vi "Run - API Logging PWP (SubVI).vi"(8 "error in (no error)":errorcluster, 10 "Elapse Time":string, 11 "Cluster":T1 {"M Event" items=["Stop", "Running", "PID", "Up Limit", "Down Limit", "Load Limit"]; "Test Type" items=["Please Select"=0, "Triaxial Shear"=1, "Triaxial UU"=2, "Shearbox"=3, "Permeability"=4, "Consolidation (Stepped Loading)/Swelling"=5, "UCT"=8, "Isotropic Consolidation"=9, "Swelling Pressure"=10, "B-Check"=11, "Saturation (Step Increment)"=12, "Saturation (Ramp)"=13]; "Data"."Test Type" items=["Please Select"=0, "Triaxial Shear"=1, "Triaxial UU"=2, "Shearbox"=3, "Permeability"=4, "Consolidation (Stepped Loading)/Swelling"=5, "UCT"=8, "Isotropic Consolidation"=9, "Swelling Pressure"=10, "B-Check"=11, "Saturation (Step Increment)"=12, "Saturation (Ramp)"=13]}) -> (0 "error out":errorcluster, 1 "JSON string":string, 2 "body":string, 3 "Cluster 2":T1 {"M Event" items=["Stop", "Running", "PID", "Up Limit", "Down Limit", "Load Limit"]; "Test Type" items=["Please Select"=0, "Triaxial Shear"=1, "Triaxial UU"=2, "Shearbox"=3, "Permeability"=4, "Consolidation (Stepped Loading)/Swelling"=5, "UCT"=8, "Isotropic Consolidation"=9, "Swelling Pressure"=10, "B-Check"=11, "Saturation (Step Increment)"=12, "Saturation (Ramp)"=13]; "Data"."Test Type" items=["Please Select"=0, "Triaxial Shear"=1, "Triaxial UU"=2, "Shearbox"=3, "Permeability"=4, "Consolidation (Stepped Loading)/Swelling"=5, "UCT"=8, "Isotropic Consolidation"=9, "Swelling Pressure"=10, "B-Check"=11, "Saturation (Step Increment)"=12, "Saturation (Ramp)"=13]})   [LabVIEW 2019]
uses:
  Controls/RunTest - Data Structure.ctl
  Controls/Test Panel - Data Structure.ctl
  Controls/Station - Test Type.ctl
  <vilib>/Utility/miscctls.llb/LVRowAndColumnTypeDef.ctl
  Controls/RunTest - Calculate Data.ctl
  <vilib>/httpClient/ClientHandle.ctl
  Controls/RunTest - Start Condition.ctl
  Controls/RunTest - Stop Condition.ctl
  Controls/UDP - Event.ctl
  <vilib>/httpClient/POSTBuffer.vi
  <vilib>/httpClient/LabVIEWHTTPClient.lvlib
panel:
  out "headers":string
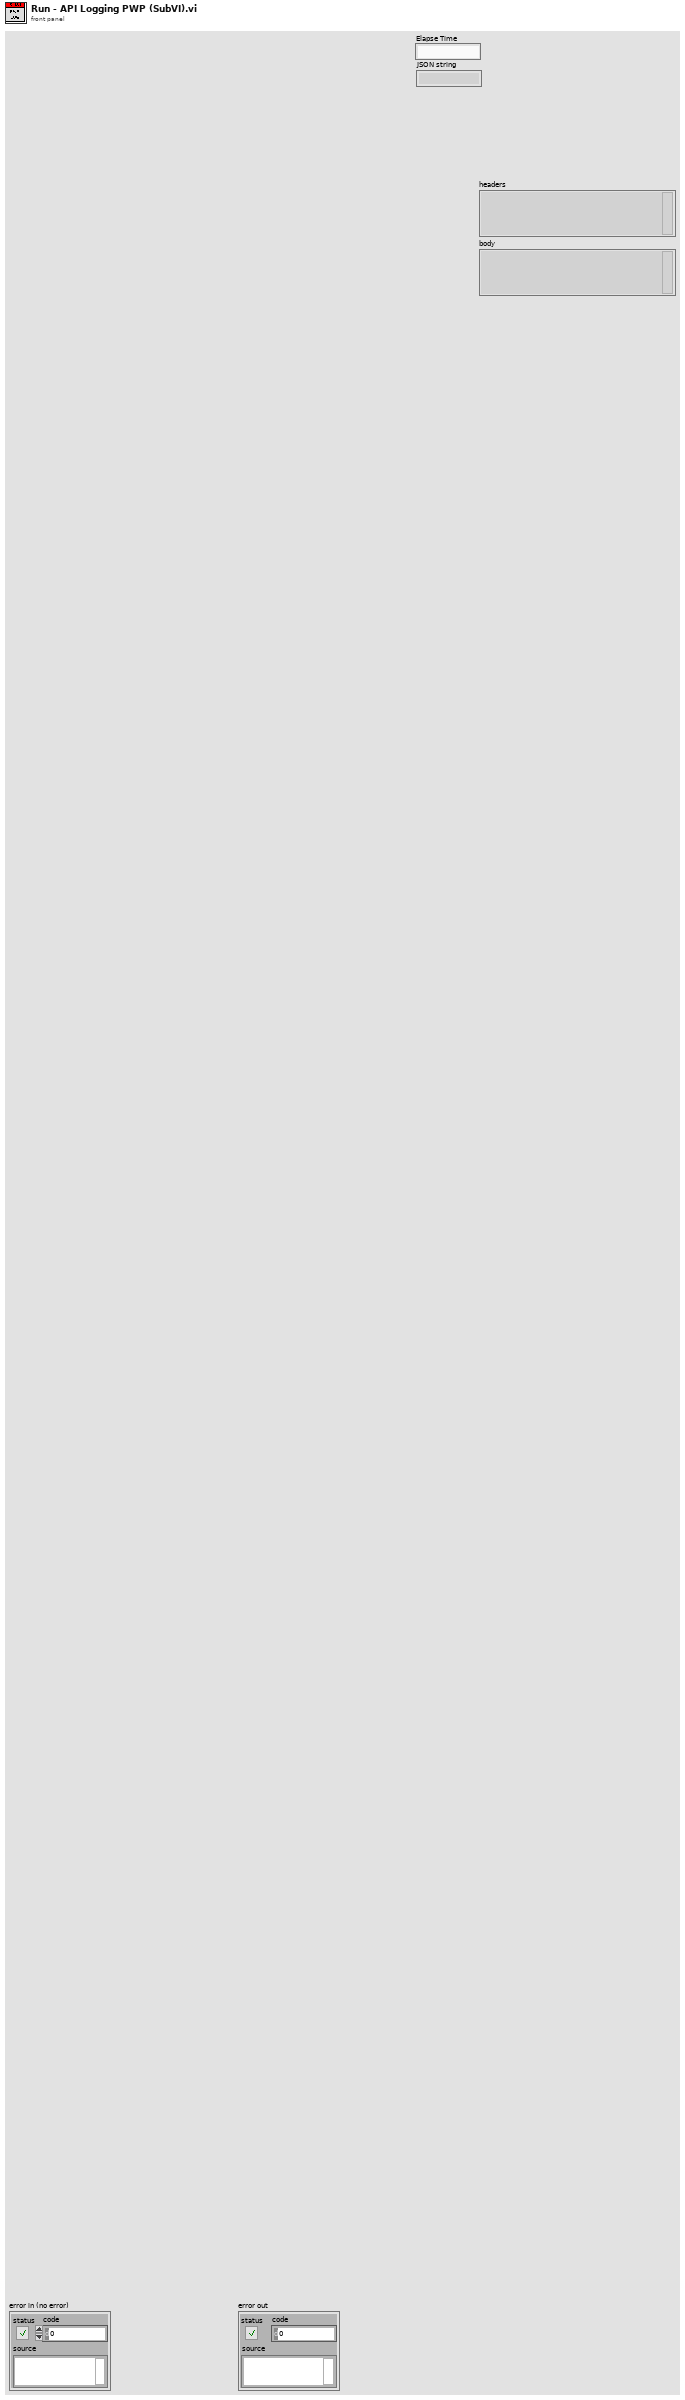
[diagram p1: front panel]
types:
  T1 = typedef "RunTest - Data Structure.ctl" = cluster{"Test Plan":string[], "PlanRow":i32, "Device Name":string[], "Timeout":i32, "Start?":bool, "Pause?":bool, "IP Address":string[], "LogRow":i32, "Logtype":u16, "Log Elapse":sgl, "Data":T2, "Stop log?":bool, "tdms":refnum<k34>, "Sensor Data":sgl[], "Start time":timestamp, "Prev Log Elapse":u32, "Plot":u16, "X-Axis":u16[], "Y-Axis":u16[], "XY":cluster{"X":dbl, "Y":dbl}[][], "End Stage?":bool, "1run":bool, "Condition":u16[], "Start Con":bool, "Log Con":bool, "Stop Con":bool, "Start Elapse":dbl, "Start Load":dbl, "Motor":i32, "StartRow":i32, "number log":i32, "Dir":bool, "Start time test":timestamp, "Auto":bool, "Check return?":bool, "Inv":cluster{"M":i32[], "Bool":bool[]}, "tdms temp":refnum<k34>, "Zero?":bool, "Plot Timer":dbl, "1st Run":bool, "TDMS Path":path, "MaxLoad":dbl, "Log Timer":sgl[], "Test Type":T3, "Log Sensor":string[], "Save?":bool, "1st Log":bool, "Y-Axis 2":u16[], "On Y-Axis 2":bool, "Decimal":u8[], "Init":cluster{"PWP TS":sgl, "Load TS":sgl, "Volume TS":sgl, "Disp TS":sgl, "CP":sgl, "Vol In":sgl, "Vol Out":sgl, "Load UCT":sgl, "Disp UCT":sgl, "PWP Sat":sgl, "CP Sat":sgl, "Volume IsoCons":sgl, "PWP IsoCons":sgl, "PWP TUU":sgl, "Load TUU":sgl, "Volume TUU":sgl, "Disp TUU":sgl, "Load Cons":sgl, "Disp Cons":sgl, "Volume Sat":sgl, "Vertical Load SB":sgl, "Vertical Disp SB":sgl, "H Disp SB":sgl, "H Load SB":sgl, "PWP BC":sgl, "CP BC":sgl, "PWP Sat Step":sgl, "CP Sat Step":sgl, "Volume Sat Step":sgl, "PWP Sat Ramp":sgl, "CP Sat Ramp":sgl, "Volume Sat Ramp":sgl}, "Calc":T5, "Device Index":i32[], "Channel Index":i32[], "http ref":T6, "fileid":string, "Step Cons":cluster{"V Stress":sgl, "H Settlement":sgl}, "RunTest":bool, "Graph Last":i32, "Init?":bool, "Datalog":bool[], "Start":T7, "Stop":T8, "Running?":bool, "StartTime":dbl, "Log Prev Time":dbl, "KeyName":string[], "Test RunTime":dbl, "Log Prev Axial":dbl, "M Event":T9[], "Last Log":bool, "popup":bool, "PreStart UU":bool, "PreStart Sat":bool, "PreStart BC":bool, "PreStart Sat Step":bool, "PreStart Sat Ramp":bool, "Prev Sat IP":string, "IP Device ID":string[]}
  T2 = typedef "Test Panel - Data Structure.ctl" = cluster{"Station":string, "Sample ID":string, "Job No":string, "Job Description":string, "Filename":string, "Test Type":T3, "Speciment No":string, "Depth":string, "Height":string, "Diameter/Length":string, "Weight":string, "Test Parameter":string, "Station[]":string[], "Edit Pos":T4, "Edit Pos Prev":T4, "Area":string, "Path":string, "sample_id":string}
  T3 = typedef "Station - Test Type.ctl" = u16
  T4 = typedef "LVRowAndColumnTypeDef.ctl" = cluster{"Row":i32, "Column":i32}
  T5 = typedef "RunTest - Calculate Data.ctl" = cluster{"TS":cluster{"Change PWP":sgl, "Change Vol":sgl, "Axial Load":sgl, "CiL":sgl, "Deviator":sgl, "Axial Strain":sgl, "MaxDeviator":sgl, "SS":sgl, "CAS":sgl}, "TUU":cluster{"Change PWP":sgl, "Axial Load":sgl, "CiL":sgl, "Deviator":sgl, "Axial Strain":sgl, "MaxDeviator":sgl}, "Sat":cluster{"B Value":sgl, "PWP Diss":sgl, "CPP":sgl, "CV":sgl}, "Per":cluster{"Change Vol In":sgl, "Change Vol Out":sgl, "Mean Vol":sgl, "Gradient Pressure":sgl, "Outlet Flow":sgl, "Inlet Flow":sgl, "I X1":sgl, "I X2":sgl, "I Y1":sgl, "I Y2":sgl, "O X1":sgl, "O X2":sgl, "O Y1":sgl, "O Y2":sgl}, "Step Cons":cluster{"V Stress":sgl, "H Settlement":sgl, "Total H Settle":sgl, "Prev Total H":sgl}, "UCT":cluster{"ALC":sgl, "H Change":sgl, "Deviator":sgl, "Axial Strain":sgl, "V Stress":sgl, "MaxDeviator":sgl}, "ISO Cons":cluster{"CPP":sgl, "PWP Diss":sgl, "CV":sgl, "VS":sgl}, "SB":cluster{"Speci LenC":sgl, "Shear Strain":sgl, "H LC":sgl, "Normal Stress":sgl, "Shear Stress":sgl, "MaxShear":sgl}, "BC":cluster{"B Value":sgl, "PWP Diss":sgl, "CPP":sgl, "CV":sgl}, "Sat Step":cluster{"B Value":sgl, "PWP Diss":sgl, "CPP":sgl, "CV":sgl}, "Sat Ramp":cluster{"B Value":sgl, "PWP Diss":sgl, "CPP":sgl, "CV":sgl}, "Prev Log":string[]}
  T6 = typedef "LabVIEWHTTPClient.lvlib/ClientHandle.ctl" = refnum<k1>
  T7 = typedef "RunTest - Start Condition.ctl" = cluster{"Cons":cluster{"VS":dbl, "Delay":bool, "No Delay":dbl}, "Sat":cluster{"CP":dbl, "BP":dbl, "StartBP":bool, "Target CP":bool, "Target BP":bool}, "Iso":cluster{"Select":dbl, "BP":dbl, "IC2":dbl, "IC3":dbl, "IC4":dbl, ". IC6":bool, "IC6":dbl, "IC6-2":dbl, "Time Cond":dbl, "Last PWP":dbl, "Target CP":bool, "Target BP":bool, "NewCP":dbl, "NewBP":dbl, "Noti CP":bool, "Noti BP":bool, "Noti PWP":bool, "PrevSatBP":dbl}, "TS":cluster{"SS":dbl, "Engage":bool, "ES":dbl, "LC":dbl, "PreStart":bool, "Trig SS":bool, "Drain":dbl, "Select":u16, "Max SS .":bool, "MaxSS":dbl}, "TUU":cluster{"SS":dbl, "Engage":bool, "ES":dbl, "LC":dbl, "PreStart":bool, "Trig SS":bool, "CP":dbl, "Delay Value":dbl, "Delay":bool, "CP PID":bool}, "UCT":cluster{"SS":dbl, "Engage":bool, "ES":dbl, "LC":dbl, "PreStart":bool, "Trig SS":bool}, "Enable?":bool, "SB":cluster{"SS":dbl, "Engage":bool, "ES":dbl, "LC":dbl, "PreStart":bool, "Trig SS":bool, "VS":dbl, "Delay Value":dbl, "Delay":bool, "VS PID":bool}, "Perm":cluster{"DP":dbl}, "BC":cluster{"CP":dbl, "Target CP":bool, "Target BP":bool, "CP Inc":dbl, "CP .Init":bool, "CP Init":dbl, "1st BC":bool}, "Sat (Step)":cluster{"Select":dbl, "CP":dbl, "BP":dbl, "EP":dbl, "StartCP":bool, "Target CP":bool, "Target BP":bool}, "Sat (Ramp)":cluster{"Select":dbl, "CP":dbl, "BP":dbl, "EP":dbl, "StartCP":bool, "Target CP":bool, "Target BP":bool, "Time Rate":u32}}
  T8 = typedef "RunTest - Stop Condition.ctl" = cluster{"Cons":cluster{"Select":i32, "Disp":dbl, "Time":dbl, "Time2":dbl, "Disp 2":dbl, "Time Cond":dbl, "Last Disp":dbl, "Swell":bool, "T50,90,100":cluster{"t50_x_min":dbl, "t50_y_value":dbl, "t90_x_min":dbl, "t90_y_value":dbl, "t100_x_min":dbl, "t100_y_value":dbl, "target_column":string, "test_type":string, "error":string}}, "Sat":cluster{"Select":i32, "PP":dbl, "Time":dbl, "VC":dbl, "Time2":dbl, "Time Cond":dbl, "Last PP":dbl, ".B":bool, "B":dbl, "Last Vc":dbl, "Time Cond 2":dbl, "Time3":dbl, "Time Cond 3":dbl, "B Achieve":bool, "PP Achieve":bool, "VC Achieve":bool, "Max Achieve":bool, "CP Check":dbl, "Skip Next":bool, "B Achieve Stage":u32, ".CP Check":bool}, "Iso":cluster{"PP":dbl, "Time":dbl, "VC":dbl, "Time2":dbl, "Time Cond":dbl, "Last Vc":dbl, ".PP":bool, "Time Cond 2":dbl, "Select":i32, "BS":cluster{"t50_x_min":dbl, "t50_y_value":dbl, "t90_x_min":dbl, "t90_y_value":dbl, "t100_x_min":dbl, "t100_y_value":dbl, "target_column":string, "test_type":string, "error":string}, "Final VC":dbl, "ASTM":cluster{"t50_x_min":dbl, "t50_y_value":dbl, "t90_x_min":dbl, "t90_y_value":dbl, "t100_x_min":dbl, "t100_y_value":dbl, "target_column":string, "test_type":string, "error":string}, "ASTM Log":cluster{"t50_x_min":dbl, "t50_y_value":dbl, "t90_x_min":dbl, "t90_y_value":dbl, "t100_x_min":dbl, "t100_y_value":dbl, "target_column":string, "test_type":string, "error":string}, "PP Achieve":bool, "VC Achieve":bool}, "TS":cluster{"Axial":dbl, ".MaxDev":bool, "MaxDev Value":dbl, "Return":bool, "Reset":bool, "Prev Time":dbl, "PostStop Run":bool, "CP Stop":bool, "BP Stop":bool, "PostStop Trig":bool, "Reset Value":dbl, "BPTrig":bool, "CPTrig":bool, "VLCTrig":bool, "CAxial":dbl, "Select":i32}, "TUU":cluster{"Axial":dbl, ".MaxDev":bool, "MaxDev Value":dbl, "Return":bool, "Reset":bool, "Prev Time":dbl, "PostStop Run":bool, "CP Stop":bool, "BP Stop":bool, "PostStop Trig":bool, "Reset Value":dbl, "BPTrig":bool, "CPTrig":bool, "VLCTrig":bool}, "UCT":cluster{"Axial":dbl, ".MaxDev":bool, "MaxDev Value":dbl, "Return":bool, "Reset":bool, "Prev Time":dbl, "PostStop Run":bool, "CP Stop":bool, "BP Stop":bool, "PostStop Trig":bool}, "Enable?":bool, "SB":cluster{"Shear":dbl, ".MaxShear":bool, "MaxShear Value":dbl, "Return":bool, "Reset":bool, "Prev Time":dbl, "PostStop Run":bool, "CP Stop":bool, "BP Stop":bool, "PostStop Trig":bool, "Reset Value":dbl, "BPTrig":bool, "CPTrig":bool, "VLCTrig":bool}, "Perm":cluster{"Max Time":bool, "Reset":bool, "PostStop Run":bool, "Ratio":bool, "Reset Value":dbl, "Time":dbl, "RatioTime":dbl, "RatioMore":dbl, "RatioLess":dbl, "Time Cond":dbl, "Time Cond 2":dbl, "Prev IF":dbl, "Prev OF":dbl, "PostStop Trig":bool, "BP Trig":bool, "DP Stop":bool, "BP Stop":bool, "CP Stop":bool, "CP Trig":bool}, "SP":cluster{".Max Time":bool, ".Time":bool, "Time":dbl, "MaxTime":dbl, "Time Cond":dbl, "Max Time Cond":dbl, "Stress":dbl}, "BC":cluster{"Select":i32, "PP":dbl, "Time":dbl, "Time Cond":dbl, "Last PP":dbl, ".B":bool, "B":dbl, "Time 2":dbl, "Time Cond 2":dbl, "B Achieve":bool, "PP Achieve":bool, "Max Achieve":bool, "CP Check":dbl, "Skip Next":bool, "B Achieve Stage":u32, ".CP Check":bool}, "Sat (Step)":cluster{"Select":i32, "PP":dbl, "Time":dbl, "VC":dbl, "Time2":dbl, "Time Cond":dbl, "Last PP":dbl, ".B":bool, "B":dbl, "Last Vc":dbl, "Time Cond 2":dbl, "Time3":dbl, "Time Cond 3":dbl, "B Achieve":bool, "PP Achieve":bool, "VC Achieve":bool, "Max Achieve":bool, "CP Check":dbl, "Skip Next":bool, "B Achieve Stage":u32}, "Sat (Ramp)":cluster{"Select":i32, "PP":dbl, "Time":dbl, "VC":dbl, "Time2":dbl, "Time Cond":dbl, "Last PP":dbl, ".B":bool, "B":dbl, "Last Vc":dbl, "Time Cond 2":dbl, "Time3":dbl, "Time Cond 3":dbl, "B Achieve":bool, "PP Achieve":bool, "VC Achieve":bool, "Max Achieve":bool, "CP Check":dbl, "Skip Next":bool, "B Achieve Stage":u32}}
  T9 = typedef "UDP - Event.ctl" = u16
  T10 = cluster{"timestamp":string, "elapsetime":string, "testname":string, "testtype":u16, "data":string[], "fileid":string, "stage":string}
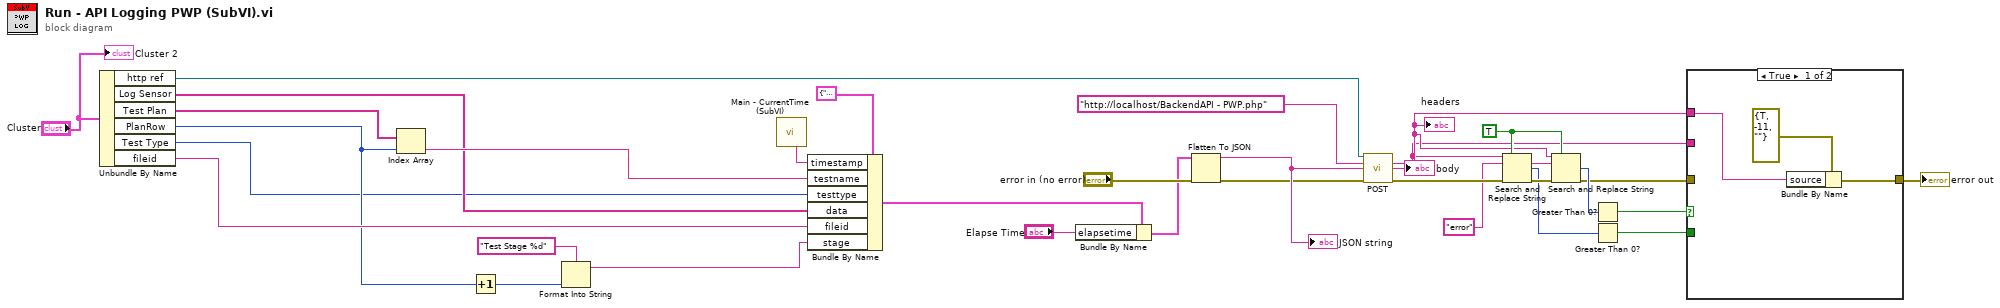
[diagram p0: block diagram]
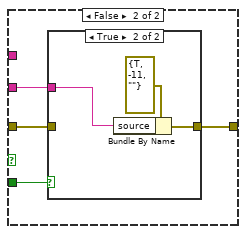
[diagram p2: hidden frame]
diagram:
  w10 = TRUE ("replace all? (F)")
  w13 = "error"
  n1 = Unbundle By Name("Cluster") -> ("http ref"=w24:T6, "Log Sensor"=w18:string[], "Test Plan"=w1:string[], "PlanRow"=w21:i32, "Test Type"=w17:T3, "fileid"=w23:string)
  n2 = Index Array(array=w1, index=w21) -> (element=w28:string)
  n3 = Increment(x=w21) -> (x+1=w20:i32)
  n4 = Format Into String(format string="Test Stage %d", w20) -> (resulting string=w19:string)  [unwired: 2 in, 1 out]
  n5 = call "Main - CurrentTime (SubVI).vi"() -> ("Time"=w16:string)  [unwired: 10 in, 1 out]
  n6 = Bundle By Name(cluster=T10 {"timestamp"="", "elapsetime"="", "testname"="", "testtype"=0, "data"=[], "fileid"="", "stage"=""}, "timestamp"=w16, "testname"=w28, "testtype"=w17, "data"=w18, "fileid"=w23, "stage"=w19) -> (w29:T10)
  n7 = Bundle By Name(cluster=w29, "elapsetime"="Elapse Time") -> (w26:T10)
  n8 = Flatten To JSON(anything=w26, error in (no error)="error in (no error)") -> (JSON string=w31:string, 11:w25:errorcluster)  [unwired: 1 in]
  "JSON string" <- w31
  n9 = call-poly <vilib>:"POST.vi"("client handle"=w24, "url"="http://localhost/BackendAPI - PWP.php", "buffer"=w31, "error in (no error)"=w25) -> ("headers"=w7:string, "body"=w4:string, "error out"=w15:errorcluster)  [unwired: 8 in, 1 out]
  "headers" <- w7
  "body" <- w4
  n10 = Search and Replace String(replace all?=w10, input string=w4, search string=w13, error in=w15) -> (number of replacements=w12:i32, error out=w14:errorcluster)  [unwired: 4 in, 2 out]
  n11 = Search and Replace String(replace all?=w10, input string=w7, search string=w13, error in=w14) -> (number of replacements=w11:i32, error out=w8:errorcluster)  [unwired: 4 in, 2 out]
  n12 = Greater Than 0?(x=w11) -> (x > 0?=w9:bool)
  n13 = Greater Than 0?(x=w12) -> (x > 0?=w5:bool)
  n14 = case shown="True" w9 {
    tunnel: w8 -> [_ w36]
    tunnel: w7 -> [w34 _]
    tunnel: [w33 w39] -> w6
    tunnel: w5 -> [_ w38]
    tunnel: w4 -> [_ w37]
    frame True {
      n15 = Bundle By Name(cluster=errorcluster {"status"=TRUE, "code"=-11, "source"=""} ("error out"), "source"=w34) -> (w33:errorcluster)
    }
    frame False {
      n16 = case shown="True" w38 {
        tunnel: w37 -> [_ w42]
        tunnel: [w40 w41] -> w39
        tunnel: w36 -> [w40 _]
        frame False {
        }
        frame True {
          n17 = Bundle By Name(cluster=errorcluster {"status"=TRUE, "code"=-11, "source"=""} ("error out"), "source"=w42) -> (w41:errorcluster)
        }
      }
    }
  }
  "error out" <- w6
  "Cluster 2" <- "Cluster"
